vi "subLoadCommandlineArgs.vi"(9 "App.Args":string[](array[string]), 11 "Options in":T1) -> (0 "error out":errorcluster, 1 "From command line?":bool, 2 "Pre-built libraries":refnum<class "ProjectItem.lvclass">[](array[class]), 3 "Options":T1, 4 "Active targets":string[](array[string]), 6 "warnings out":errorcluster)   [LabVIEW 2019, in "SolutionBuilder.lvlib" / "SolutionBuilder.lvclass"]
uses:
  SolutionBuilder.lvclass
  Options.ctl
  ProjectItem/ProjectItem.lvclass
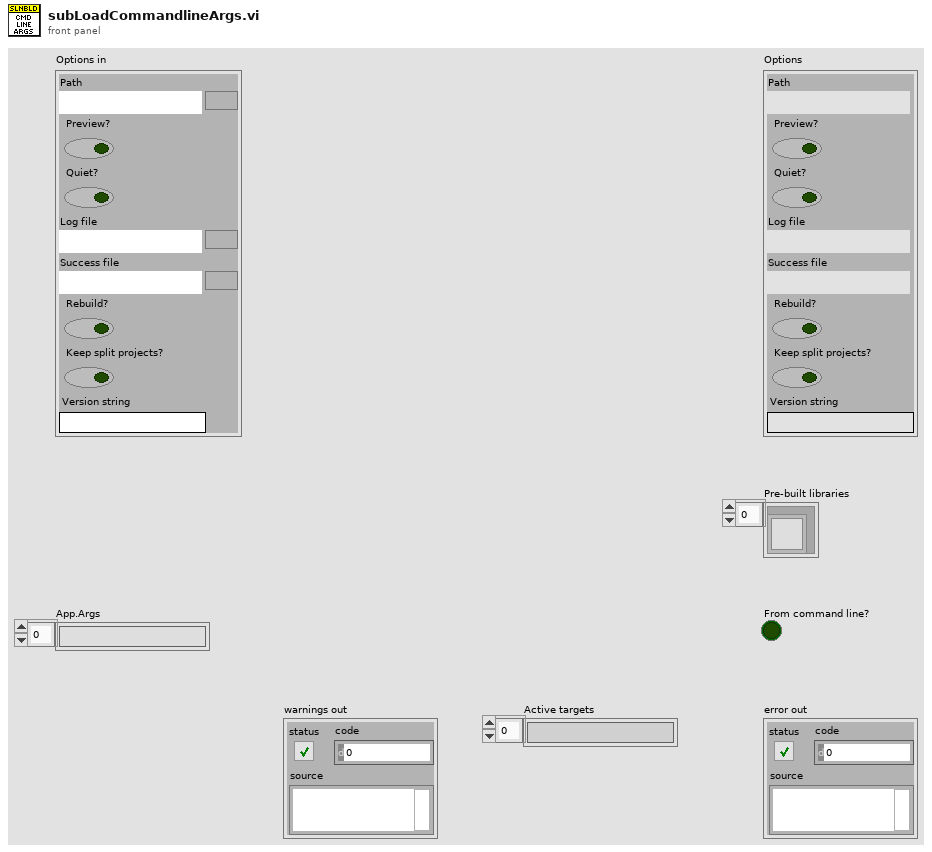
[diagram p1: front panel]
types:
  T1 = typedef "SolutionBuilder.lvlib/SolutionBuilder.lvclass/Options.ctl" = cluster{"Path":path, "Preview?":bool, "Quiet?":bool, "Log file":path, "Success file":path, "Rebuild?":bool, "Keep split projects?":bool, "Version string":string}
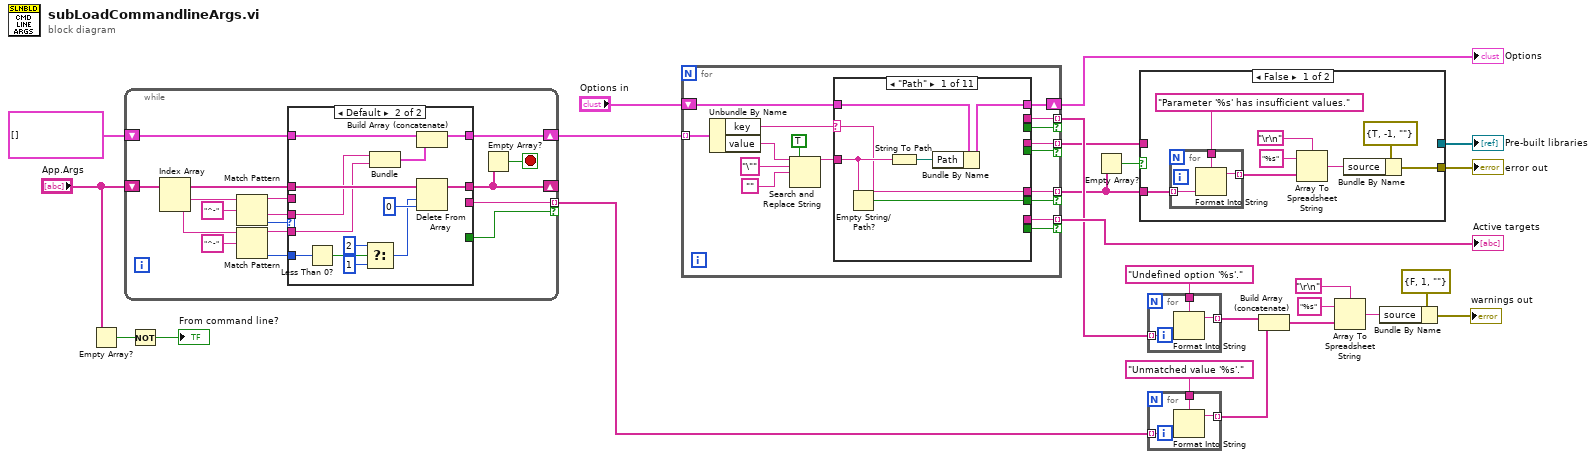
[diagram p0: block diagram]
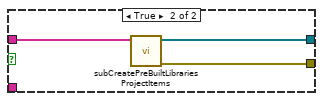
[diagram p2: hidden frame]
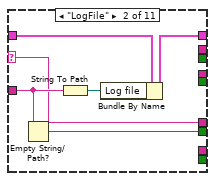
[diagram p3: hidden frame]
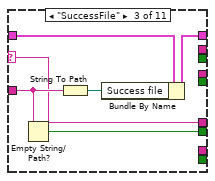
[diagram p4: hidden frame]
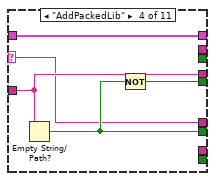
[diagram p5: hidden frame]
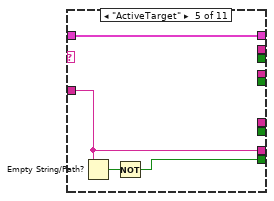
[diagram p6: hidden frame]
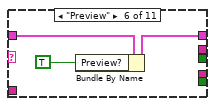
[diagram p7: hidden frame]
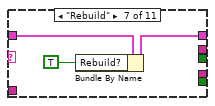
[diagram p8: hidden frame]
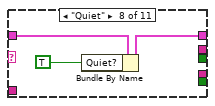
[diagram p9: hidden frame]
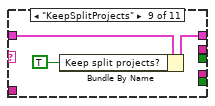
[diagram p10: hidden frame]
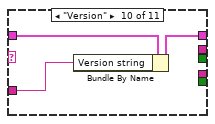
[diagram p11: hidden frame]
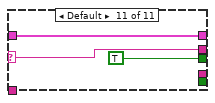
[diagram p12: hidden frame]
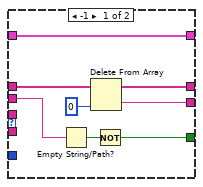
[diagram p13: hidden frame]
diagram:
  n1 = Empty Array?(array="App.Args") -> (empty?=w25:bool)
  n2 = while {
    shift-right: [w30] -> _
    shift-left: "App.Args" -> [w33]
    shift-right: [w31] -> w22
    shift-left: cluster{"key":string, "value":string}[] [] -> [w32]
    tunnel: [w28] -> w15 mode=indexing if=w27
    stop <- w29 stop-if-true
    n3 = Index Array(array=w33) -> (element #1=w41:string, element #2=w38:string)  [unwired: 2 in]
    n4 = Match Pattern(string=w41, regular expression="^-") -> (before substring=w26:string, after substring=w36:string, offset past match=w37:i32)  [unwired: 1 in, 1 out]
    n5 = Match Pattern(string=w38, regular expression="^-") -> (before substring=w35:string, offset past match=w34:i32)  [unwired: 1 in, 2 out]
    n6 = case shown="Default" w37 {
      tunnel: w36 -> [_ w54]
      tunnel: w35 -> [_ w53]
      tunnel: w34 -> [_ w62]
      tunnel: w33 -> [w48 w60]
      tunnel: [w47 w55] -> w30
      tunnel: w32 -> [w46 w52]
      tunnel: [w46 w50] -> w31
      tunnel: [w45 _] -> w28
      tunnel: [w42 _] -> w27
      tunnel: w26 -> [w44 _]
      frame -1 {
        n7 = Empty String/Path?(string/path=w44) -> (empty?=w43:bool)
        n8 = Delete From Array(array=w48, index=0) -> (deleted portion=w45:string, array with subset deleted=w47:string[])  [unwired: 1 in]
        n9 = Not(x=w43) -> (.not. x?=w42:bool)
      }
      frame Default {
        n10 = Less Than 0?(x=w62) -> (x < 0?=w61:bool)
        n11 = Select(t=2 ("length"), s=w61, f=1 ("length")) -> (s? t:f=w56:i32)
        n12 = Bundle(w54, w53) -> (w51:cluster{string, string})  [unwired: 1 in]
        n13 = Build Array (concatenate)(w52, w51) -> (w50:cluster{string, string}[])
        n14 = Delete From Array(array=w60, length=w56, index=0) -> (array with subset deleted=w55:string[])  [unwired: 1 out]
      }
    }
    n15 = Empty Array?(array=w30) -> (empty?=w29:bool)
  }
  n16 = Not(x=w25) -> (.not. x?=→"From command line?":bool)
  n17 = for {
    shift-right: [w78] -> w21
    shift-left: "Options in" -> [w79]
    tunnel: w22 -> [w77] mode=indexing
    tunnel: [w75] -> w14 mode=indexing if=w74
    tunnel: [w73] -> w16 mode=indexing if=w72
    tunnel: [w71] -> w1 mode=indexing if=w70
    tunnel: [w69] -> w20 mode=indexing if=w68
    n18 = Unbundle By Name(w77) -> ("key"=w76:string, "value"=w67:string)
    n19 = Search and Replace String(replace all?=TRUE ("replace all? (F)"), input string=w67, search string="\"", replace string="") -> (result string=w66:string)  [unwired: 4 in, 3 out]
    n20 = case shown="\"Path\"" w76 {
      selector: w76 -> [w81 w87 w93 w99 _ _ _ _ _ _ w123]
      tunnel: w79 -> [w85 w91 w97 w102 w106 w109 w112 w115 w118 w121 w124]
      tunnel: w66 -> [w82 w88 w94 w101 w104 _ _ _ _ w119 _]
      tunnel: [w84 w90 w96 w102 w106 w108 w111 w114 w117 w120 w124] -> w78
      tunnel: [_ _ _ w101 _ _ _ _ _ _ _] -> w75
      tunnel: [_ _ _ w98 _ _ _ _ _ _ _] -> w74
      tunnel: [_ _ _ _ _ _ _ _ _ _ w123] -> w73
      tunnel: [_ _ _ _ _ _ _ _ _ _ TRUE] -> w72
      tunnel: [w81 w87 w93 w99 _ _ _ _ _ _ _] -> w71
      tunnel: [w80 w86 w92 w100 _ _ _ _ _ _ _] -> w70
      tunnel: [_ _ _ _ w104 _ _ _ _ _ _] -> w69
      tunnel: [_ _ _ _ w103 _ _ _ _ _ _] -> w68
      frame "Path" {
        n21 = Empty String/Path?(string/path=w82) -> (empty?=w80:bool)
        n22 = String To Path(string=w82) -> (path=w83:path)
        n23 = Bundle By Name(cluster=w85, "Path"=w83) -> (w84:T1)
      }
      frame "LogFile" {
        n24 = Empty String/Path?(string/path=w88) -> (empty?=w86:bool)
        n25 = String To Path(string=w88) -> (path=w89:path)
        n26 = Bundle By Name(cluster=w91, "Log file"=w89) -> (w90:T1)
      }
      frame "SuccessFile" {
        n27 = Empty String/Path?(string/path=w94) -> (empty?=w92:bool)
        n28 = String To Path(string=w94) -> (path=w95:path)
        n29 = Bundle By Name(cluster=w97, "Success file"=w95) -> (w96:T1)
      }
      frame "AddPackedLib" {
        n30 = Empty String/Path?(string/path=w101) -> (empty?=w100:bool)
        n31 = Not(x=w100) -> (.not. x?=w98:bool)
      }
      frame "ActiveTarget" {
        n32 = Empty String/Path?(string/path=w104) -> (empty?=w105:bool)
        n33 = Not(x=w105) -> (.not. x?=w103:bool)
      }
      frame "Preview" {
        n34 = Bundle By Name(cluster=w109, "Preview?"=TRUE) -> (w108:T1)
      }
      frame "Rebuild" {
        n35 = Bundle By Name(cluster=w112, "Rebuild?"=TRUE ("Preview?")) -> (w111:T1)
      }
      frame "Quiet" {
        n36 = Bundle By Name(cluster=w115, "Quiet?"=TRUE ("Preview?")) -> (w114:T1)
      }
      frame "KeepSplitProjects" {
        n37 = Bundle By Name(cluster=w118, "Keep split projects?"=TRUE ("Preview?")) -> (w117:T1)
      }
      frame "Version" {
        n38 = Bundle By Name(cluster=w121, "Version string"=w119) -> (w120:T1)
      }
      frame Default {
      }
    }
  }
  "Options" <- w21
  "Active targets" <- w20
  n39 = Empty Array?(array=w1) -> (empty?=w2:bool)
  n40 = case shown="False" w2 {
    tunnel: w14 -> [_ w138]
    tunnel: [_ w137] -> w13
    tunnel: [w125 w136] -> w12
    tunnel: w1 -> [w132 _]
    frame False {
      n41 = for {
        tunnel: w132 -> [w135] mode=indexing
        tunnel: [w134] -> w126 mode=indexing
        tunnel: "Parameter '%s' has insufficient values." ("format string") -> [w133]
        n42 = Format Into String(format string=w133, w135) -> (resulting string=w134:string)  [unwired: 2 in, 1 out]
      }
      n43 = Array To Spreadsheet String(delimiter (Tab)="\r\n", array=w126, 3:"%s" ("format string")) -> (spreadsheet string=w130:string)
      n44 = Bundle By Name(cluster=errorcluster {"status"=TRUE, "code"=-1, "source"=""} ("error out"), "source"=w130) -> (w125:errorcluster)
    }
    frame True {
      n45 = call "subCreatePreBuiltLibrariesProjectItems.vi"("Lib definition strings"=w138) -> ("error out"=w136:errorcluster, "Pre-built libraries"=w137:refnum<class "ProjectItem.lvclass">[])  [unwired: 9 in]
    }
  }
  "error out" <- w12
  "Pre-built libraries" <- w13
  n46 = for {
    tunnel: w16 -> [w141] mode=indexing
    tunnel: [w140] -> w6 mode=indexing
    tunnel: "Undefined option '%s'." ("format string") -> [w139]
    n47 = Format Into String(format string=w139, w141) -> (resulting string=w140:string)  [unwired: 2 in, 1 out]
  }
  n48 = for {
    tunnel: w15 -> [w144] mode=indexing
    tunnel: [w143] -> w4 mode=indexing
    tunnel: "Unmatched value '%s'." ("format string") -> [w142]
    n49 = Format Into String(format string=w142, w144) -> (resulting string=w143:string)  [unwired: 2 in, 1 out]
  }
  n50 = Build Array (concatenate)(w6, w4) -> (w5:string[])
  n51 = Array To Spreadsheet String(delimiter (Tab)="\r\n", array=w5, 3:"%s" ("format string")) -> (spreadsheet string=w8:string)
  n52 = Bundle By Name(cluster=errorcluster {"status"=FALSE, "code"=1, "source"=""} ("error out"), "source"=w8) -> (→"warnings out":errorcluster)
